vi "G_Paths.vi"() -> ()   [LabVIEW 2021, in "Channel.lvlib"]
uses:
  Channel.lvlib
panel:
  in  "ChannelsFile":path
  in  "Plugins Folder":path
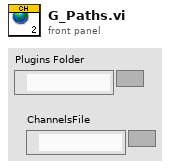
[diagram p1: front panel]
diagram:
